vi "Measurement Logic.vi"() -> ()   [LabVIEW 2021, in "NIDCPowerSourceDCVoltage.lvlib"]
uses:
  NIDCPowerSourceDCVoltage.lvlib
  Measurement Configuration.ctl
  Measurement Results.ctl
  <vilib>/Plug-In SDKs/Measurements/Measure Call Context/Measure Call Context.lvclass
  <vilib>/Plug-In SDKs/Clients/Session Management V1/Session Reservation/Session Reservation.lvclass
  <vilib>/Plug-In SDKs/Sessions/niDCPower/NI Session Management niDCPower.lvlib
panel:
  out "measure call context out":refnum<class "Measure Call Context.lvclass">
  in  "measure call context in":refnum<class "Measure Call Context.lvclass">
  out "measurement results":T1
  in  "measurement configuration":T2={"pin_names"=[], "voltage_level"=6.0, "voltage_level_range"=6.0, "current_limit"=0.01, "current_limit_range"=0.01, "source_delay"=0.0}
  out "error out":errorcluster
  in  "error in":errorcluster
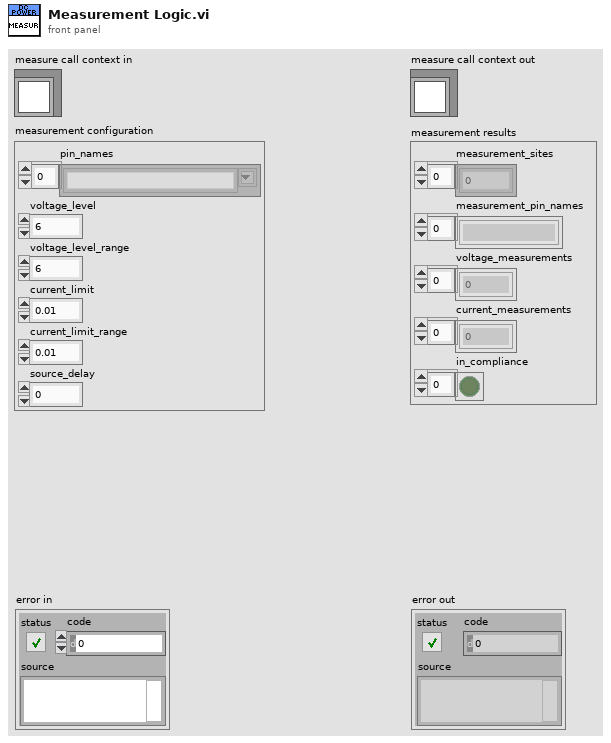
[diagram p1: front panel]
types:
  T1 = typedef "NIDCPowerSourceDCVoltage.lvlib/Measurement Results.ctl" = cluster{"measurement_sites":i32[], "measurement_pin_names":string[], "voltage_measurements":dbl[], "current_measurements":dbl[], "in_compliance":bool[]}
  T2 = typedef "NIDCPowerSourceDCVoltage.lvlib/Measurement Configuration.ctl" = cluster{"pin_names":string[], "voltage_level":dbl, "voltage_level_range":dbl, "current_limit":dbl, "current_limit_range":dbl, "source_delay":dbl}
  T3 = typedef "NI Session Management niDCPower.lvlib/Connection with Session.ctl" = cluster{"connection":T4, "session":refnum<k15>}
  T4 = typedef "NI Session Management V1 Client.lvlib/Session Reservation.lvclass/Connection.ctl" = cluster{"pin or relay name":string, "site":i32, "instrument type id":string, "channel":string}
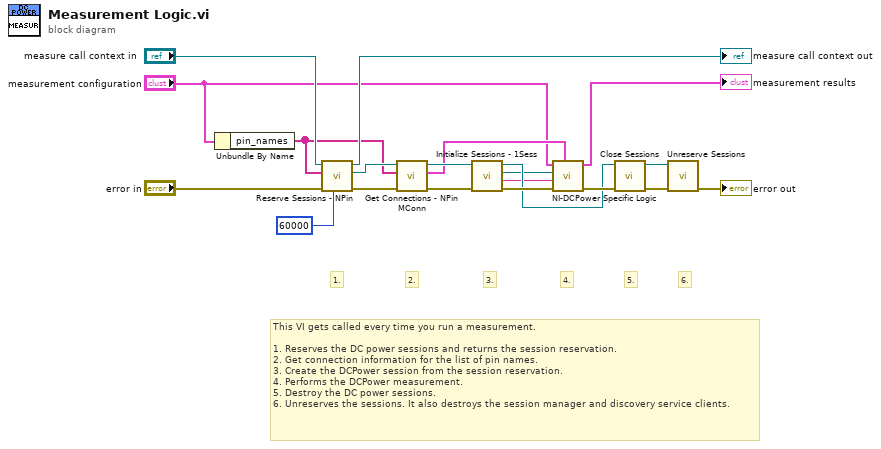
[diagram p0: block diagram]
diagram:
  # "6."
  # "This VI gets called every time you run a measurement.\n\n1. Reserves the DC power sessions and returns the session reservation.\n2. Get connection information for the list of pin names.\n3. Create the DCPower session from the session reservation.\n4. Performs the DCPower measurement.\n5. Destroy the DC power sessions.\n6. Unreserves the sessions. It also destroys the session manager and discovery service clients."
  # "5."
  # "4."
  # "3."
  # "2."
  # "1."
  n1 = Unbundle By Name("measurement configuration") -> ("pin_names"=w7:string[])
  n2 = call <vilib>:"Reserve Sessions - NPin.vi"("timeout (ms)"=60000, "error in"="error in", "pin or relay names"=w7, "measurement context in"="measure call context in") -> ("error out"=w10:errorcluster, "session reservation out"=w8:refnum<class "Session Reservation.lvclass">, "measurement context out"=→"measure call context out":refnum<class "Measure Call Context.lvclass">)  [unwired: 5 in]
  n3 = call <vilib>:"Get Connections - NPin MConn.vi"("error in"=w10, "pin or relay names"=w7, "session reservation in"=w8) -> ("error out"=w9:errorcluster, "connections"=w5:T3[], "session reservation out"=w6:refnum<class "Session Reservation.lvclass">)  [unwired: 6 in]
  n4 = call <vilib>:"Initialize Sessions - 1Sess.vi"("error in"=w9, "session reservation in"=w6) -> ("error out"=w19:errorcluster, "channel list"=w3:string, "session"=w4:refnum<k15>, "session reservation out"=w14:refnum<class "Session Reservation.lvclass">)  [unwired: 6 in]
  n5 = call "NI-DCPower Specific Logic.vi"("connections"=w5, "error in"=w19, "channel list"=w3, "instrument handle"=w4, "Measurement Configuration"="measurement configuration") -> ("error out"=w18:errorcluster, "Measurement Results"=→"measurement results":T1)  [unwired: 4 in, 1 out]
  n6 = call <vilib>:"Close Sessions.vi"("error in"=w18, "session reservation in"=w14) -> ("error out"=w17:errorcluster, "session reservation out"=w15:refnum<class "Session Reservation.lvclass">)  [unwired: 8 in]
  n7 = call <vilib>:"Unreserve Sessions.vi"("error in"=w17, "session reservation in"=w15) -> ("error out"=→"error out":errorcluster)  [unwired: 9 in]
